vi "RFH-align_data.vi"(7 "Xi":dbl[](array[numeric]), 10 "Common Format":T1) -> (2 "Common Format alligned":T1)   [LabVIEW 2020, in "RFH-Reflection_File_Handler.lvlib"]
doc: "Interpolates every array of a Common Format cluster onto the frequencies Xi."
uses:
  RFH-Reflection_File_Handler.lvlib
  RFH-common_data_format.ctl
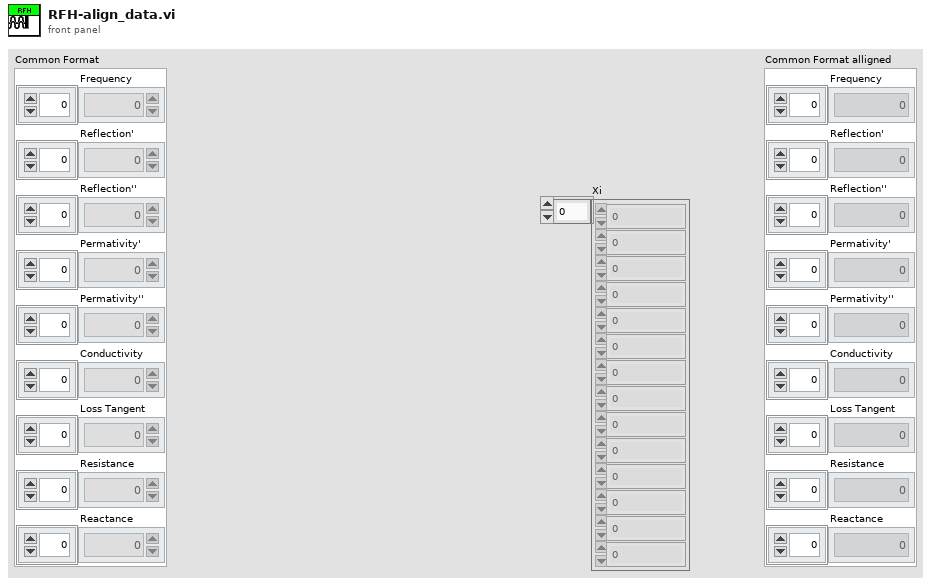
[diagram p1: front panel]
types:
  T1 = typedef "RFH-Reflection_File_Handler.lvlib/RFH-common_data_format.ctl" = cluster{"Frequency":dbl[], "Reflection'":dbl[], "Reflection''":dbl[], "Permativity'":dbl[], "Permativity''":dbl[], "Conductivity":dbl[], "Loss Tangent":dbl[], "Resistance":dbl[], "Reactance":dbl[]}
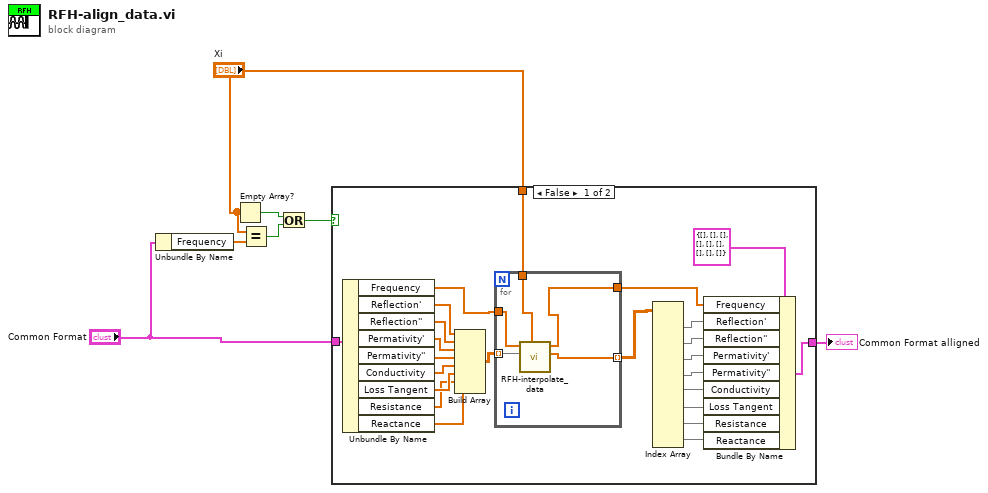
[diagram p0: block diagram]
diagram:
  n1 = Unbundle By Name("Common Format") -> ("Frequency"=w2:dbl[])
  n2 = Empty Array?(array="Xi") -> (empty?=w6:bool)
  n3 = Equal?(x="Xi", y=w2) -> (x = y?=w1:bool)
  n4 = Or(x=w6, y=w1) -> (x .or. y?=w5:bool)
  n5 = case shown="False" w5 {
    tunnel: "Xi" -> [w27 _]
    tunnel: "Common Format" -> [w26 w37]
    tunnel: [w19 w37] -> w7
    frame False {
      n6 = Unbundle By Name(w26) -> ("Frequency"=w28:dbl[], "Reflection'"=w31:dbl[], "Reflection''"=w30:dbl[], "Permativity'"=w18:dbl[], "Permativity''"=w17:dbl[], "Conductivity"=w15:dbl[], "Loss Tangent"=w14:dbl[], "Resistance"=w11:dbl[], "Reactance"=w10:dbl[])
      n7 = Build Array(w31, w30, w18, w17, w15, w14, w11, w10) -> (w29:dbl[][])
      n8 = for {
        tunnel: w29 -> [w36] mode=indexing
        tunnel: w28 -> [w35]
        tunnel: w27 -> [w34]
        tunnel: [w32] -> w21 mode=indexing
        tunnel: [w33] -> w20
        n9 = call "RFH-interpolate_data.vi"("Xi"=w34, "data"=w36, "Frequency"=w35) -> ("data out"=w32:dbl[], "Frequency out"=w33:dbl[])  [unwired: 7 in]
      }
      n10 = Index Array(array=w21) -> (element #1=w22:dbl[], element #2=w23:dbl[], element #3=w24:dbl[], element #4=w25:dbl[], element #5=w13:dbl[], element #6=w12:dbl[], element #7=w8:dbl[], element #8=w9:dbl[])  [unwired: 16 in]
      n11 = Bundle By Name(cluster=T1 {"Frequency"=[], "Reflection'"=[], "Reflection''"=[], "Permativity'"=[], "Permativity''"=[], "Conductivity"=[], "Loss Tangent"=[], "Resistance"=[], "Reactance"=[]} ("Common Format"), "Frequency"=w20, "Reflection'"=w22, "Reflection''"=w23, "Permativity'"=w24, "Permativity''"=w25, "Conductivity"=w13, "Loss Tangent"=w12, "Resistance"=w8, "Reactance"=w9) -> (w19:T1)
    }
    frame True {
    }
  }
  "Common Format alligned" <- w7
